vi "laser_single_current_output.vi"(7 "Laser Active":bool, 8 "error in":errorcluster, 10 "Current":cluster{"Value":dbl, "Units":dbl}={"Value"=0.0, "Units"=0.001} {"Units" items=["mA"=0.001, "A"=1.0]}, 11 "VISA resource name":refnum<visa-resource-name>) -> (0 "error out":errorcluster, 3 "VISA resource name out":refnum<visa-resource-name>)   [LabVIEW 2025, in "tSNIP.lvlib"]
uses:
  tSNIP.lvlib
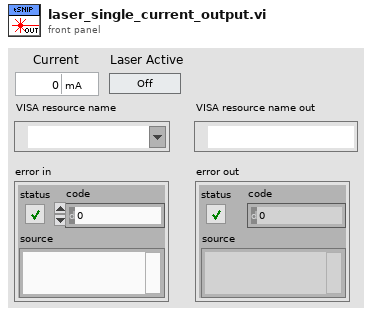
[diagram p1: front panel]
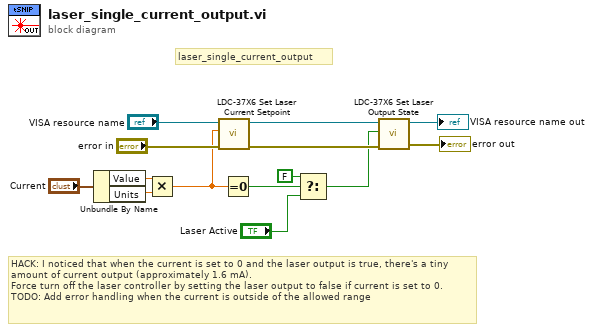
[diagram p0: block diagram]
diagram:
  # "laser_single_current_output"
  # "HACK: I noticed that when the current is set to 0 and the laser output is true, there's a tiny amount of current output (approximately 1.6 mA).\nForce turn off the laser controller by setting the laser output to false if current is set to 0.\nTODO: Add error handling when the current is outside of the allowed range"
  n1 = Unbundle By Name("Current") -> ("Value"=w11:dbl, "Units"=w7:dbl)
  n2 = Multiply(x=w11, y=w7) -> (x*y=w6:dbl)
  n3 = call <instrlib>:"LDC-37X6 Set Laser Current Setpoint.vi"("error in"="error in", "Laser Current Setpoint (A)"=w6, "VISA resource name"="VISA resource name") -> ("error out"=w13:errorcluster, "VISA resource name out"=w14:refnum<visa-resource-name>)  [unwired: 7 in]
  n4 = Equal To 0?(x=w6) -> (x = 0?=w4:bool)
  n5 = Select(t=FALSE, s=w4, f="Laser Active") -> (s? t:f=w2:bool)
  n6 = call <instrlib>:"LDC-37X6 Set Laser Output State.vi"("error in"=w13, "Laser Output Enable"=w2, "VISA resource name"=w14) -> ("error out"=→"error out":errorcluster, "VISA resource name out"=→"VISA resource name out":refnum<visa-resource-name>)  [unwired: 7 in]
